vi "mupExpr Calc.vi"() -> ()   [LabVIEW 2015]
uses:
  mupExpr/mupExpr.lvclass
  mupExpr/mupExpr.lvclass/mupExpr.ctl
  mupExpr/Eval_SglRes.vi
  mupLib/mupEval.vi
  mupLib/mupCheckError.vi
  <vilib>/Utility/error.llb/Error Cluster From Error Code.vi
panel:
  out "Result":dbl=nan format="%#_20g"
  in  "Expression":string="0"
  in  "Calculate":bool
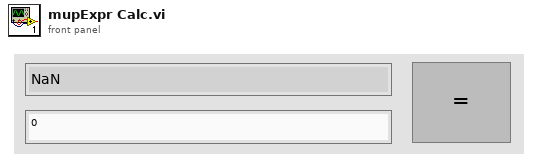
[diagram p1: front panel]
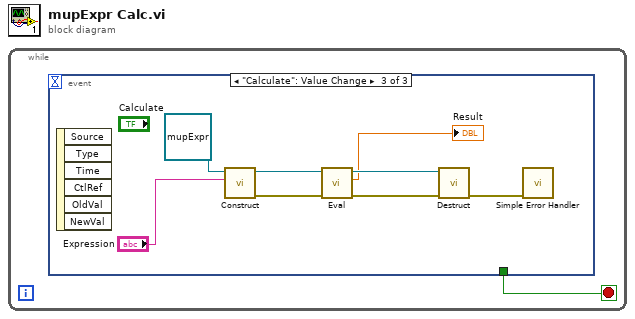
[diagram p0: block diagram]
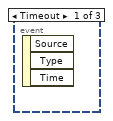
[diagram p2: hidden frame]
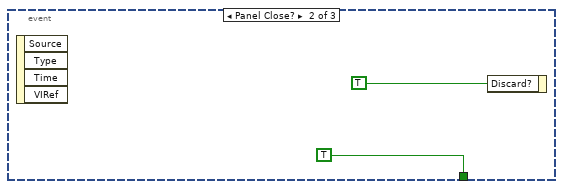
[diagram p3: hidden frame]
diagram:
  n1 = while {
    stop <- w1 stop-if-true
    n2 = event shown="[2] \"Calculate\": Value Change" {
      selector: _ -> [_ _ _]
      dyn-events: _ -> [_ _ _]
      timeout: _ -> [_ _ _]
      tunnel: [_ TRUE _] -> w1
      event Timeout {
        n3 = event-data() -> ()  [unwired: 1 in, 3 out]
      }
      event Panel Close? {
        n4 = event-data() -> ()  [unwired: 1 in, 4 out]
        n5 = event-data("Discard?"=TRUE) -> ()  [unwired: 1 in, 1 out]
      }
      event "Calculate": Value Change {
        n6 = event-data() -> ()  [unwired: 1 in, 6 out]
        n7 = call-dynamic "Construct.vi"("Expression"="Expression", "muExpr in"=refnum<class "mupExpr.lvclass"> refnum) -> ("error out"=w10:errorcluster, "mupExpr out"=w8:refnum<class "mupExpr.lvclass">)  [unwired: 6 in, 2 out]
        n8 = call-poly "Eval.vi"("error in (no error)"=w10, "muExpr in"=w8) -> ("error out"=w11:errorcluster, "Result"=→"Result":dbl, "muExpr out"=w9:refnum<class "mupExpr.lvclass">)  [unwired: 7 in]
        n9 = call-dynamic "Destruct.vi"("error in (no error)"=w11, "muExpr in"=w9) -> ("error out"=w5:errorcluster)  [unwired: 9 in]
        n10 = call <vilib>:"Simple Error Handler.vi"("error in (no error)"=w5) -> ()  [unwired: 4 in, 5 out]
      }
    }
  }
